vi "After Each.vi"(8 "Error In":errorcluster, 11 "Writer In":refnum<class "Writer.lvclass">) -> (0 "Error Out":errorcluster, 3 "Data":string)   [LabVIEW 2018, in "Tests.lvlib" / "Writer.lvlib"]
uses:
  Writer.lvlib
  src/Toolkit/Public/Writer/Writer.lvclass
  src/Toolkit/Public/Writer/Private/End by Value.vi
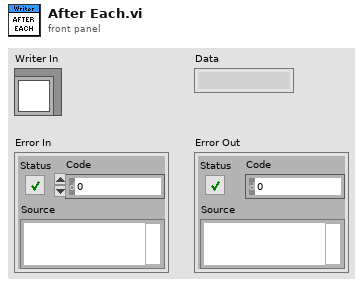
[diagram p1: front panel]
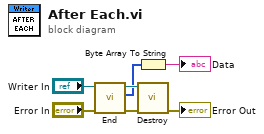
[diagram p0: block diagram]
diagram:
  n1 = call-poly "End.vi"("Error In"="Error In", "Writer In"="Writer In") -> ("Error Out"=w2:errorcluster, "Data"=w1:u8[], "Writer Out"=w3:refnum<class "Writer.lvclass">)  [unwired: 7 in]
  n2 = Byte Array To String(unsigned byte array=w1) -> (string=→"Data":string)
  n3 = call "Destroy.vi"("Error In"=w2, "Writer"=w3) -> ("Error Out"=→"Error Out":errorcluster)  [unwired: 9 in]
